vi "VIH HelpGen - Get VI Conpane Control Refnums.vi"(7 "Sort terminals (T)":bool=TRUE, 8 "error in":errorcluster, 11 "VI Reference":refnum<vi>) -> (0 "error out":errorcluster, 1 "Ctrl Attributes":T1[](array[typedef]), 2 "Conpane Ctrl Refnums":refnum<vi>[](array[refnum]), 3 "dup VI Reference":refnum<vi>)   [LabVIEW 2014]
doc: "::: VI Helpeks :::\nCopyright (c) 2000-2026 Konstantin Shifershteyn. All rights reserved."
uses:
  VIH HelpGen Typedef - Control Terminal Attributes Cluster.ctl
panel:
  # "VI Helpeks\nCopyright (c) 2012-2026 Konstantin Shifershteyn"
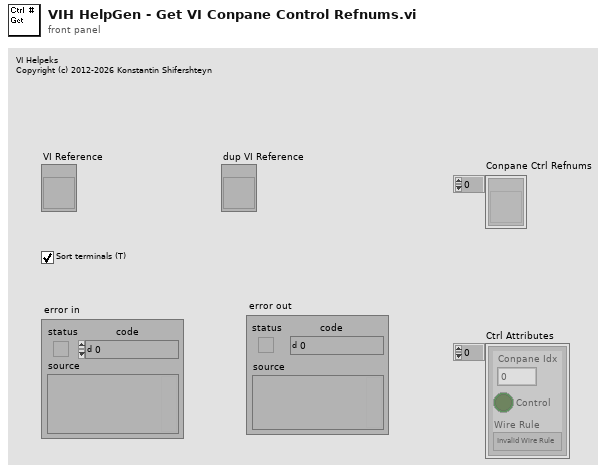
[diagram p1: front panel]
types:
  T1 = typedef "VIH HelpGen Typedef - Control Terminal Attributes Cluster.ctl" = cluster{"Conpane Idx":i32, "Control":bool, "Wire Rule":enum16{"Invalid Wire Rule", "Required", "Recommended", "Optional", "Dynamic Dispatch"}}
  T2 = typedef "LVRectTypeDef.ctl" = cluster{"Left":i16, "Top":i16, "Right":i16, "Bottom":i16}
  T3 = enum16{"Invalid Wire Rule", "Required", "Recommended", "Optional", "Dynamic Dispatch"}[]
  T4 = enum16{"Invalid Wire Rule", "Required", "Recommended", "Optional", "Dynamic Dispatch"}
  T5 = cluster{"Indicator":bool, "Bottom":i16, "Left":i16, i32}
  T6 = cluster{"Indicator":bool, "Bottom":i16, "Left":i16, i32}[]
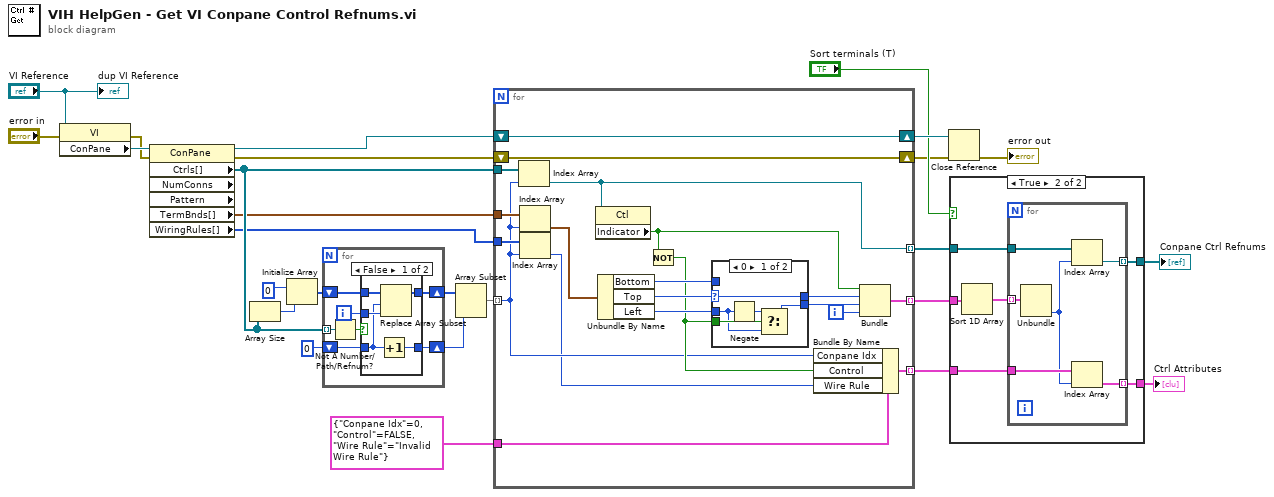
[diagram p0: block diagram]
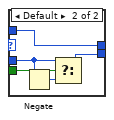
[diagram p4: hidden frame]
diagram:
  n1 = property class="VI"(reference="VI Reference", error in="error in") -> (error out=w11:errorcluster, "ConPane"=w17:refnum<vi>)  [unwired: 1 out]
  n2 = property class="ConPane" props=["Ctrls[]", "NumConns", "Pattern", "TermBnds[]", "WiringRules[]"](reference=w17, error in=w11) -> (reference out=w26:refnum<vi>, error out=w7:errorcluster, "Ctrls[]"=w18:refnum<vi>[], "TermBnds[]"=w15:T2[], "WiringRules[]"=w2:T3)  [unwired: 2 out]
  n3 = Array Size(array=w18) -> (size(s)=w20:i32)
  n4 = Initialize Array(0, w20) -> (w19:i32[])
  n5 = for {
    shift-right: [w32] -> w23
    shift-left: w19 -> [w33]
    shift-right: [w30] -> w22
    shift-left: 0 -> [w31]
    tunnel: w18 -> [w27] mode=indexing
    i -> [w29]
    n6 = Not A Number/Path/Refnum?(number/path/refnum=w27) -> (NaN/Path/Refnum?=w28:bool)
    n7 = case shown="False" w28 {
      tunnel: w33 -> [w38 w40]
      tunnel: [w37 w40] -> w32
      tunnel: w29 -> [w36 _]
      tunnel: w31 -> [w35 w39]
      tunnel: [w34 w39] -> w30
      frame False {
        n8 = Increment(x=w35) -> (x+1=w34:i32)
        n9 = Replace Array Subset(array=w38, new element=w36, index=w35) -> (w37:i32[])
      }
      frame True {
      }
    }
  }
  n10 = Array Subset(array=w23, length=w22) -> (w16:i32[])  [unwired: 1 in]
  n11 = for {
    tunnel: w18 -> [w59]
    shift-right: [w60] -> w25
    shift-left: w26 -> [w60]
    tunnel: w16 -> [w43] mode=indexing
    tunnel: w15 -> [w58]
    tunnel: [w55] -> w14 mode=indexing
    tunnel: [w54] -> w13 mode=indexing
    shift-right: [w46] -> w6
    shift-left: w7 -> [w46]
    tunnel: [w45] -> w4 mode=indexing
    tunnel: w2 -> [w44]
    tunnel: T1 {"Conpane Idx"=0, "Control"=FALSE, "Wire Rule"=enum."Invalid Wire Rule"} -> [w41]
    i -> [w56]
    n12 = Index Array(array=w59, index=w43) -> (element=w45:refnum<vi>)
    n13 = Index Array(array=w58, index=w43) -> (element=w57:T2)
    n14 = Index Array(array=w44, index=w43) -> (element=w42:T4)
    n15 = property class="Ctl"(reference=w45) -> ("Indicator"=w47:bool)  [unwired: 1 in, 2 out]
    n16 = Unbundle By Name(w57) -> ("Bottom"=w49:i16, "Top"=w53:i16, "Left"=w51:i16)
    n17 = Not(x=w47) -> (.not. x?=w48:bool)
    n18 = case shown="0" w53 {
      selector: w53 -> [w65 _]
      tunnel: [w65 w66] -> w52
      tunnel: w48 -> [w64 w67]
      tunnel: w51 -> [w63 w69]
      tunnel: [w61 w70] -> w50
      tunnel: w49 -> [_ w66]
      frame 0 {
        n19 = Negate(x=w63) -> (-x=w62:i16)
        n20 = Select(t=w62, s=w64, f=w63) -> (s? t:f=w61:i16)
      }
      frame Default {
        n21 = Negate(x=w69) -> (-x=w68:i16)
        n22 = Select(t=w69, s=w67, f=w68) -> (s? t:f=w70:i16)
      }
    }
    n23 = Bundle By Name(cluster=w41, "Conpane Idx"=w43, "Control"=w48, "Wire Rule"=w42) -> (w54:T1)
    n24 = Bundle("Indicator"=w47, "Bottom"=w52, "Left"=w50, w56) -> (w55:T5)  [unwired: 1 in]
  }
  n25 = Close Reference(reference=w25, error in (no error)=w6) -> (error out=→"error out":errorcluster)
  n26 = case shown="True" "Sort terminals (T)" {
    tunnel: w14 -> [_ w78]
    tunnel: w13 -> [w72 w76]
    tunnel: [w72 w75] -> w5
    tunnel: w4 -> [w71 w74]
    tunnel: [w71 w73] -> w3
    frame False {
    }
    frame True {
      n27 = Sort 1D Array(array=w78) -> (sorted array=w77:T6)
      n28 = for {
        tunnel: w77 -> [w84] mode=indexing
        tunnel: w76 -> [w83]
        tunnel: [w82] -> w75 mode=indexing
        tunnel: w74 -> [w81]
        tunnel: [w79] -> w73 mode=indexing
        n29 = Unbundle(w84) -> (w80:i32)  [unwired: 3 out]
        n30 = Index Array(array=w81, index=w80) -> (element=w79:refnum<vi>)
        n31 = Index Array(array=w83, index=w80) -> (element=w82:T1)
      }
    }
  }
  "Ctrl Attributes" <- w5
  "Conpane Ctrl Refnums" <- w3
  "dup VI Reference" <- "VI Reference"
